vi "CD Add Channel.vi"(8 "error in":errorcluster, 11 "Node Ptr":T1 format="%.0x") -> (0 "error out":errorcluster)   [LabVIEW 2017, in "PXImc System Explorer.lvlib"]
uses:
  PXImc System Explorer.lvlib
  <vilib>/NI Veristand/Custom Device API/Custom Device Item Ref.ctl
  Shared/Channel.ctl
  <vilib>/NI Veristand/Custom Device API/Custom Device Channel Type.ctl
  <vilib>/NI VeriStand/Custom Device API/Custom Device API.lvlib
  Shared/PXImc Shared.lvlib
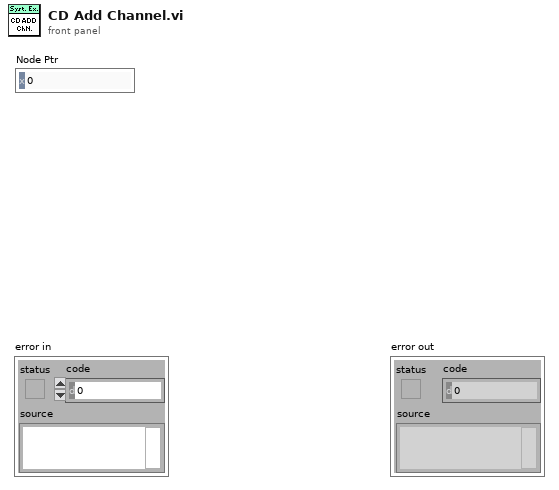
[diagram p1: front panel]
types:
  T1 = typedef "Custom Device API.lvlib/Custom Device Item Ref.ctl" = u64
  T2 = typedef "PXImc Shared.lvlib/Channel.ctl" = cluster{"Name":string, "Units":string, "Default":dbl, "Description":string}
  T3 = typedef "Custom Device API.lvlib/Custom Device Channel Type.ctl" = enum16{"Input", "Output"}
  T4 = typedef "Custom Device API.lvlib/Custom Device Item Info.ctl" = cluster{"Name":string, "Is Channel":bool, "GUID":string, "Is Waveform":bool}
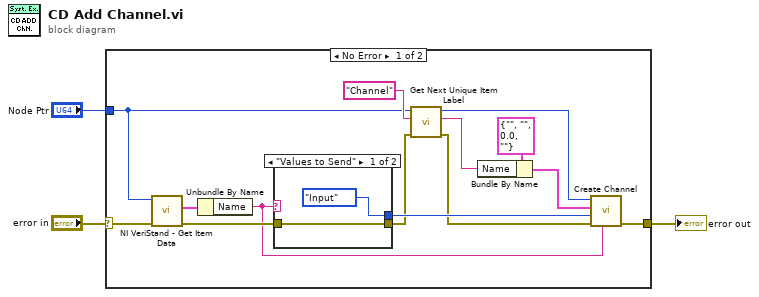
[diagram p0: block diagram]
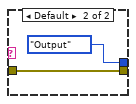
[diagram p2: hidden frame]
diagram:
  n1 = case shown="No Error" "error in" {
    selector: "error in" -> [w15 w22]
    tunnel: [w17 w22] -> w2
    tunnel: "Node Ptr" -> [w6 _]
    frame No Error {
      n2 = call <vilib>:"NI VeriStand - Get Item Data.vi"("error in (no error)"=w15, "Item Ref in"=w6) -> ("error out"=w14:errorcluster, "Item Info"=w16:T4)  [unwired: 6 in, 2 out]
      n3 = Unbundle By Name(w16) -> ("Name"=w5:string)
      n4 = case shown="\"Values to Send\"" w5 {
        tunnel: [w19 w21] -> w9
        tunnel: w14 -> [w19 w21]
        tunnel: [Custom_Device_Channel_Type."Input" ("Type") Custom_Device_Channel_Type."Output" ("Type")] -> w13
        frame "Values to Send" {
        }
        frame Default {
        }
      }
      n5 = call "Get Next Unique Item Label.vi"("error in (no error)"=w9, "Label"="Channel" ("string"), "Parent Ref in"=w6) -> ("error out"=w8:errorcluster, "Label out"=w4:string, "Parent Ref dup"=w7:T1)  [unwired: 5 in, 1 out]
      n6 = Bundle By Name(cluster=T2 {"Name"="", "Units"="", "Default"=0.0, "Description"=""} ("Channel"), "Name"=w4) -> (w11:T2)
      n7 = call "Create Channel.vi"("New Section Name (none)"=w5, "error in"=w8, "Type"=w13, "Channel"=w11, "Item Ref in"=w7) -> ("error out"=w17:errorcluster)  [unwired: 5 in, 1 out]
    }
    frame Error {
    }
  }
  "error out" <- w2
